vi "BMS UI.vi"() -> ()   [LabVIEW 2020]
uses:
  <vilib>/Instr/_visa.llb/VISA Configure Serial Port (Instr).vi
panel:
  out "BALANCING":bool
  out "LOAD":bool
  out "SETTING":bool
  out "Voltage Max (mV)":dbl=3.741
  out "Voltage Min (mV)":dbl=3.635
  out "Temperature (C)":dbl=27.0
  out "Current (A)":dbl
  out "SOC (%)":dbl=56.7
  out "Total Voltage (V)":dbl=36.816
  in  "Tab Control":T1(tab)=enum."Cell Voltage"
  out "Total Voltage":dbl(graph)=56.7
  out "SOC":dbl(graph)=56.7
  out "Current":dbl(graph)
  out "Temperature":dbl(graph)=27.0
  out "Cell Voltage":i32[][](graph)=[[3714, 3717, 3726, 3710, 3741, 3639, 3641, 3635, 3641, 3652, 0, 0, 0, 0, 0]]
  out "Delta Voltage":i32(graph)
  out "Cell 2":i32(slide)=3717 scale=0.0..4300.0
  out "Cell 15":i32(slide) scale=0.0..4300.0
  out "Cell 14":i32(slide) scale=0.0..4300.0
  out "Cell 13":i32(slide) scale=0.0..4300.0
  out "Cell 12":i32(slide) scale=0.0..4300.0
  out "Cell 11":i32(slide) scale=0.0..4300.0
  out "Cell 10":i32(slide)=3652 scale=0.0..4300.0
  out "Cell 9":i32(slide)=3641 scale=0.0..4300.0
  out "Cell 8":i32(slide)=3635 scale=0.0..4300.0
  out "Cell 7":i32(slide)=3641 scale=0.0..4300.0
  out "Cell 6":i32(slide)=3639 scale=0.0..4300.0
  out "Cell 5":i32(slide)=3741 scale=0.0..4300.0
  out "Cell 4":i32(slide)=3710 scale=0.0..4300.0
  out "Cell 3":i32(slide)=3726 scale=0.0..4300.0
  out "Cell 1":i32(slide)=3714 scale=0.0..4300.0
  out "Data Receive":string="36816,567,0,270,3635,3741,106,0,0,0,3714,3717,3726,3710,3741,3639,3641,3635,3641,3652,0,0,0,0,0\n"
  in  "stop":bool
  in  "BAUND RATE":u32=115200
  in  "PORT":refnum<visa-resource-name>="COM5"
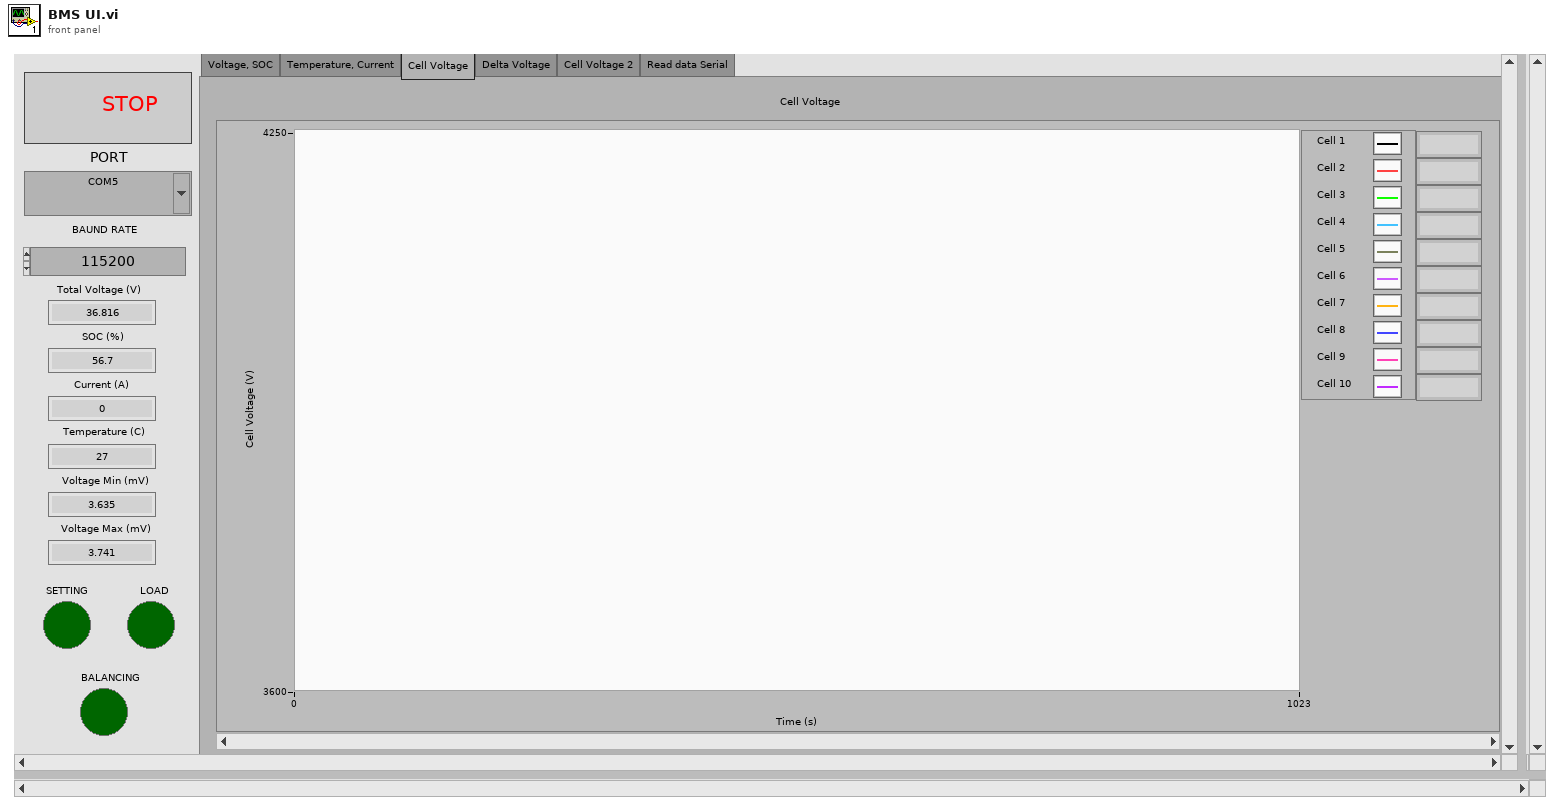
[diagram p1: front panel]
types:
  T1 = enum32{"Voltage, SOC", "Temperature, Current", "Cell Voltage", "Delta Voltage", "Cell Voltage 2", "Read data Serial"}
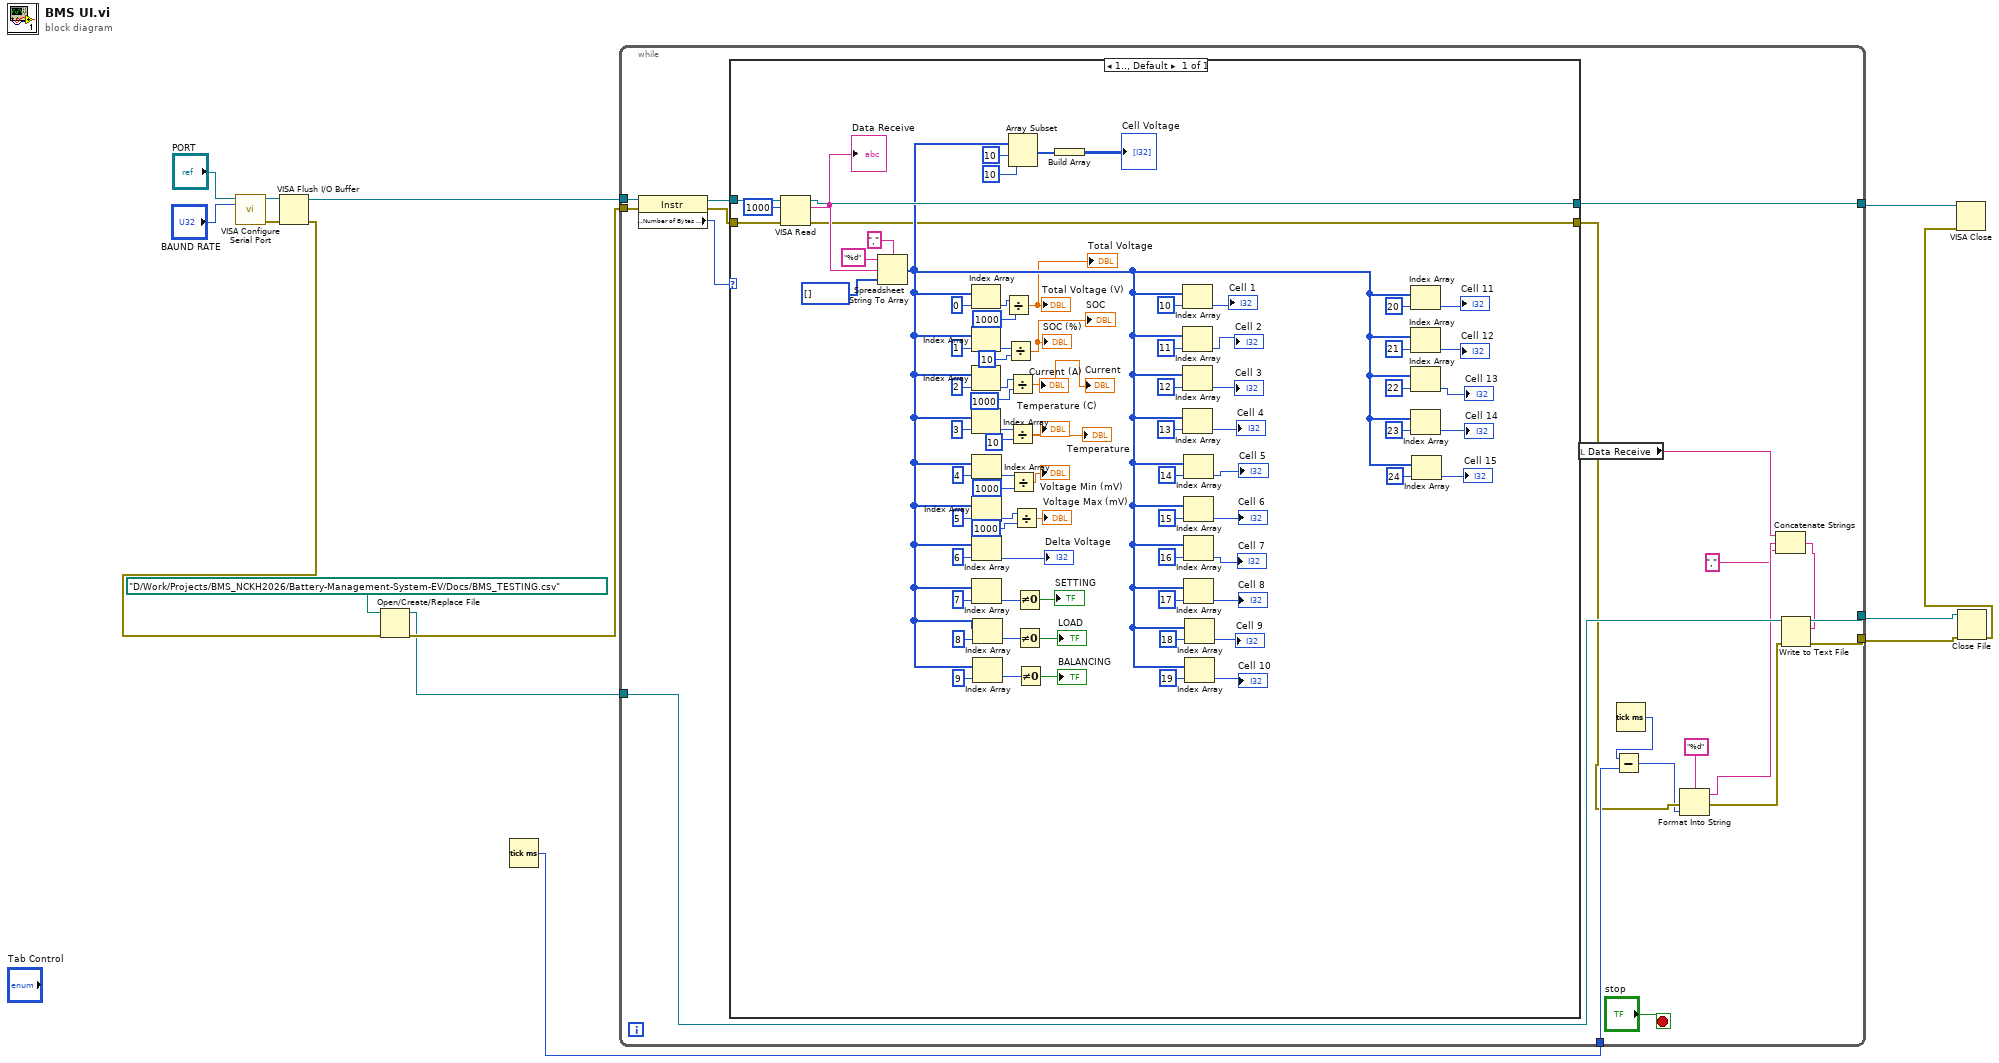
[diagram p0: block diagram]
diagram:
  n1 = call-poly "VISA Configure Serial Port"("VISA resource name"="PORT", "baud rate (9600)"="BAUND RATE") -> ("VISA resource name out"=w11:refnum<visa-resource-name>, "error out"=w12:errorcluster)  [unwired: 12 in]
  n2 = VISA Flush I/O Buffer(VISA resource name=w11, error in (no error)=w12) -> (VISA resource name out=w10:refnum<visa-resource-name>, error out=w4:errorcluster)  [unwired: 1 in]
  n3 = Open/Create/Replace File(file path (use dialog)=path "D:/Work/Projects/BMS_NCKH2026/Battery-Management-System-EV/Docs/BMS_TESTING.csv", error in=w4) -> (refnum out=w2:refnum<file>, error out=w3:errorcluster)  [unwired: 4 in, 1 out]
  n4 = Tick Count (ms)() -> (millisecond timer value=w1:u32)
  n5 = while {
    tunnel: w10 -> [w33]
    tunnel: w3 -> [w32]
    tunnel: [w28] -> w9
    tunnel: [w25] -> w7
    tunnel: [w26] -> w8
    tunnel: w2 -> [w27]
    tunnel: w1 -> [w21]
    stop <- "stop" stop-if-true
    n6 = property class="Instr"(reference=w33, error in=w32) -> (reference out=w30:refnum<visa-resource-name>, error out=w29:errorcluster, "Serial Settings:Number of Bytes at Serial Port"=w31:u32)
    n7 = case shown="1.., Default" w31 {
      tunnel: w30 -> [w113]
      tunnel: w29 -> [w112]
      tunnel: [w110] -> w28
      tunnel: [w36] -> w19
      frame 1.., Default {
        n8 = VISA Read(VISA resource name=w113, byte count=u32 1000, error in (no error)=w112) -> (VISA resource name out=w110:refnum<visa-resource-name>, read buffer=w109:string, error out=w36:errorcluster)  [unwired: 1 out]
        "Data Receive" <- w109
        n9 = Spreadsheet String To Array(delimiter (Tab)=",", format string="%d", spreadsheet string=w109, array type (2D Dbl)=i32[] []) -> (array=w55:i32[])
        n10 = Index Array(array=w55, index=0) -> (element=w66:i32)
        n11 = Index Array(array=w55, index=1) -> (element=w40:i32)
        n12 = Index Array(array=w55, index=2) -> (element=w64:i32)
        n13 = Index Array(array=w55, index=3) -> (element=w43:i32)
        n14 = Index Array(array=w55, index=4) -> (element=w62:i32)
        n15 = Index Array(array=w55, index=5) -> (element=w60:i32)
        n16 = Index Array(array=w55, index=6) -> (element=→"Delta Voltage":i32)
        n17 = Index Array(array=w55, index=7) -> (element=w49:i32)
        n18 = Index Array(array=w55, index=8) -> (element=w46:i32)
        n19 = Index Array(array=w55, index=9) -> (element=w45:i32)
        n20 = Divide(x=w66, y=1000) -> (x/y=→"Total Voltage (V)" →"Total Voltage":dbl)
        n21 = Divide(x=w40, y=10) -> (x/y=→"SOC (%)" →"SOC":dbl)
        n22 = Array Subset(array=w55, index=10, length=10) -> (w51:i32[])
        n23 = Divide(x=w64, y=1000) -> (x/y=→"Current (A)" →"Current":dbl)
        n24 = Divide(x=w43, y=10) -> (x/y=→"Temperature (C)" →"Temperature":dbl)
        n25 = Divide(x=w62, y=1000) -> (x/y=→"Voltage Min (mV)":dbl)
        n26 = Divide(x=w60, y=1000) -> (x/y=→"Voltage Max (mV)":dbl)
        n27 = Not Equal To 0?(x=w49) -> (x != 0?=→"SETTING":bool)
        n28 = Not Equal To 0?(x=w46) -> (x != 0?=→"LOAD":bool)
        n29 = Not Equal To 0?(x=w45) -> (x != 0?=→"BALANCING":bool)
        n30 = Build Array(w51) -> (→"Cell Voltage":i32[][])
        n31 = Index Array(array=w55, index=10) -> (element=→"Cell 1":i32)
        n32 = Index Array(array=w55, index=11) -> (element=→"Cell 2":i32)
        n33 = Index Array(array=w55, index=12) -> (element=→"Cell 3":i32)
        n34 = Index Array(array=w55, index=13) -> (element=→"Cell 4":i32)
        n35 = Index Array(array=w55, index=14) -> (element=→"Cell 5":i32)
        n36 = Index Array(array=w55, index=15) -> (element=→"Cell 6":i32)
        n37 = Index Array(array=w55, index=16) -> (element=→"Cell 7":i32)
        n38 = Index Array(array=w55, index=17) -> (element=→"Cell 8":i32)
        n39 = Index Array(array=w55, index=18) -> (element=→"Cell 9":i32)
        n40 = Index Array(array=w55, index=19) -> (element=→"Cell 10":i32)
        n41 = Index Array(array=w55, index=20) -> (element=→"Cell 11":i32)
        n42 = Index Array(array=w55, index=21) -> (element=→"Cell 12":i32)
        n43 = Index Array(array=w55, index=22) -> (element=→"Cell 13":i32)
        n44 = Index Array(array=w55, index=23) -> (element=→"Cell 14":i32)
        n45 = Index Array(array=w55, index=24) -> (element=→"Cell 15":i32)
      }
    }
    n46 = local read "Data Receive"() -> (w24:string)
    n47 = Tick Count (ms)() -> (millisecond timer value=w22:u32)
    n48 = Subtract(x=w22, y=w21) -> (x-y=w15:u32)
    n49 = Format Into String(format string="%d", error in=w19, w15) -> (resulting string=w17:string, error out=w18:errorcluster)  [unwired: 1 in]
    n50 = Concatenate Strings(w24, w17, "," ("string")) -> (w23:string)
    n51 = Write to Text File(file (use dialog)=w27, text=w23, error in=w18) -> (refnum out=w25:refnum<file>, error out=w26:errorcluster)  [unwired: 1 in, 1 out]
  }
  n52 = Close File(refnum=w7, error in=w8) -> (error out=w6:errorcluster)  [unwired: 1 out]
  n53 = VISA Close(VISA resource name=w9, error in (no error)=w6) -> ()  [unwired: 1 out]
